vi "Add Process to Map.vi"(8 "error in (no error)":errorcluster, 10 "Process Out":refnum<class "Process.lvclass">, 11 "Application In":refnum<class "Application.lvclass">) -> (0 "error out":errorcluster, 3 "Application Out":refnum<class "Application.lvclass">)   [LabVIEW 2020, in "Application.lvclass"]
uses:
  Application.lvclass
  Process/Process.lvclass
  Application.lvclass/Application.ctl
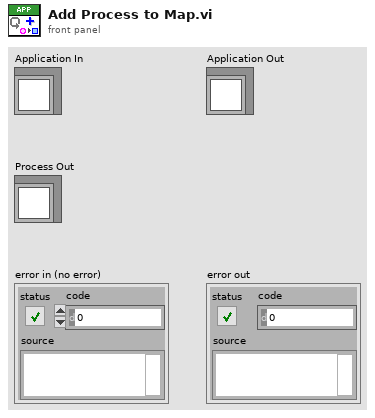
[diagram p1: front panel]
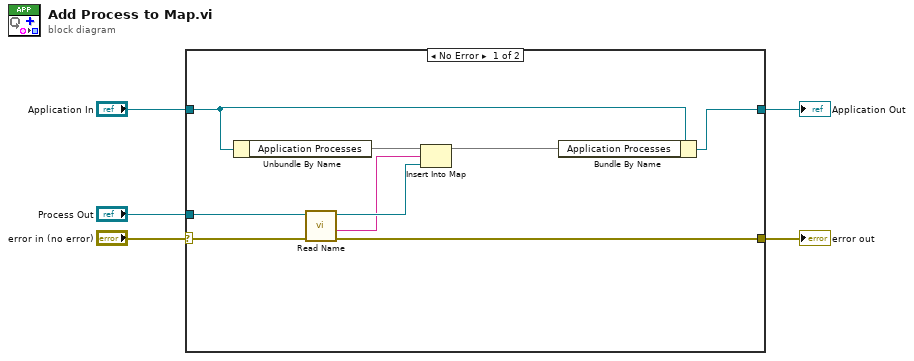
[diagram p0: block diagram]
diagram:
  n1 = case shown="No Error" "error in (no error)" {
    selector: "error in (no error)" -> [w14 w15]
    tunnel: [w13 w16] -> w4
    tunnel: "Process Out" -> [w11 _]
    tunnel: "Application In" -> [w10 w16]
    tunnel: [w6 w15] -> w1
    frame No Error {
      n2 = Unbundle By Name(w10) -> ("Application Processes"=w8:map{string, refnum<class "Process.lvclass">})
      n3 = call "Read Name.vi"("error in (no error)"=w14, "Process In"=w11) -> ("error out"=w6:errorcluster, "Name"=w7:string, "Process Out"=w9:refnum<class "Process.lvclass">)  [unwired: 6 in, 1 out]
      n4 = Insert Into Map(map in=w8, key=w7, value=w9) -> (map out=w12:map{string, refnum<class "Process.lvclass">})  [unwired: 2 out]
      n5 = Bundle By Name(cluster=w10, "Application Processes"=w12) -> (w13:refnum<class "Application.lvclass">)
    }
    frame Error {
    }
  }
  "error out" <- w1
  "Application Out" <- w4
